vi "Test MQTT-3.3.2-3.vi"(8 "error in (no error)":errorcluster, 11 "Connection Config":refnum<class "Connection.lvclass">) -> (0 "error out":errorcluster, 3 "Connection Config dup":refnum<class "Connection.lvclass">)   [LabVIEW 2013]
uses:
  <vilib>/LabVIEW Open Source Project/MQTT Connection/MQTT_Connection/Connection/Connection.lvclass
  <vilib>/LabVIEW Open Source Project/MQTT Client/Client class/Client.lvclass/Client.ctl
  <vilib>/LabVIEW Open Source Project/MQTT Control Packets/Control Packets/PUBLISH/PUBLISH.lvclass
  <vilib>/addons/_JKI Toolkits/Caraya/classes/Test/Test.lvclass
  <vilib>/LabVIEW Open Source Project/MQTT Client/Client class/Client.lvclass
  <vilib>/addons/_JKI Toolkits/Caraya/classes/Assert/Assert.lvclass
  <vilib>/LabVIEW Open Source Project/MQTT Connection/MQTT_Base/Base Class/MQTT_Base.lvclass
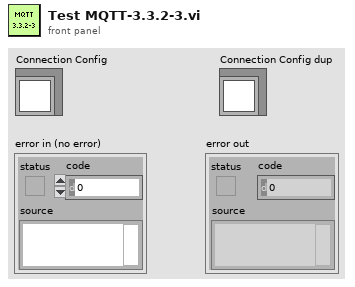
[diagram p1: front panel]
types:
  T1 = typedef "MQTT Client.lvlib/Client.lvclass/Public Events -- cluster.ctl" = cluster{"Connection Status":refnum<user-event>, "Connected":refnum<user-event>, "Application Message":refnum<user-event>}
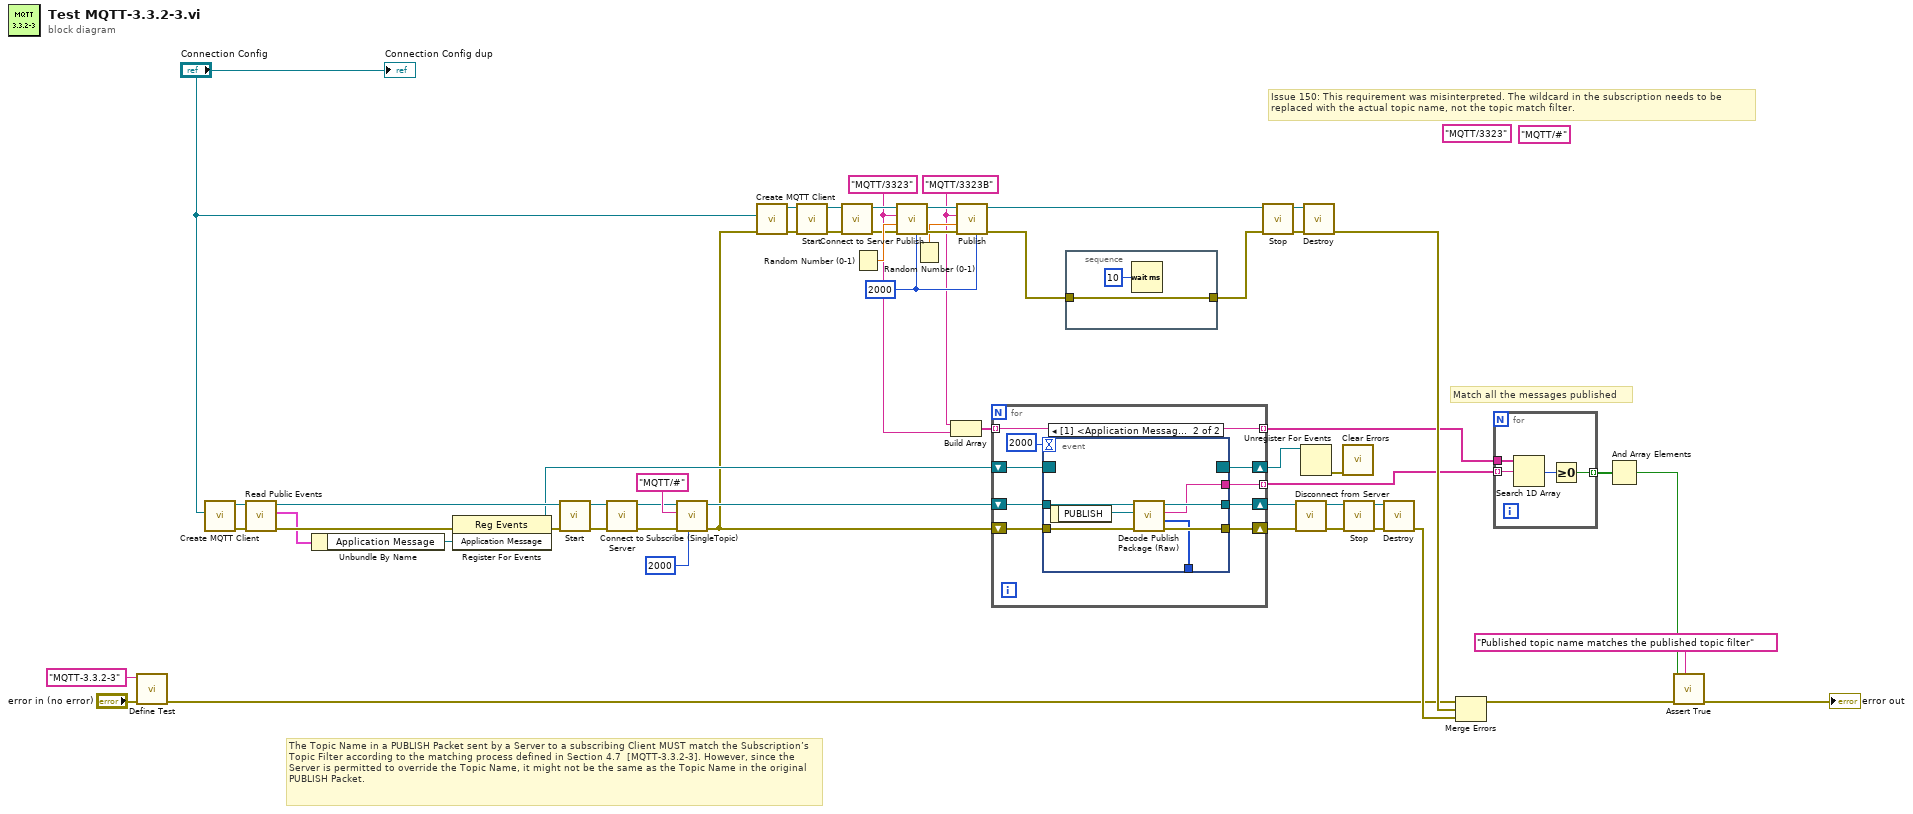
[diagram p0: block diagram]
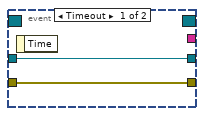
[diagram p2: hidden frame]
diagram:
  w36 = 2000 ("timeout (100ms)")
  w11 = "MQTT/3323B" ("Topic Filter")
  (unwired) "MQTT/3323" ("Topic Filter")
  (unwired) "MQTT/#" ("Topic Filter")
  w10 = "MQTT/3323" ("Topic Filter")
  # "Match all the messages published"
  # "Issue 150: This requirement was misinterpreted. The wildcard in the subscription needs to be\nreplaced with the actual topic name, not the topic match filter."
  # "The Topic Name in a PUBLISH Packet sent by a Server to a subscribing Client MUST match the Subscription’s Topic Filter according to the matching process defined in Section 4.7  [MQTT-3.3.2-3]. However, since the Server is permitted to override the Topic Name, it might not be the same as the Topic Name in the original PUBLISH Packet."
  n1 = call <vilib>:"Define Test.vi"("error in (no error)"="error in (no error)", "Label (VI Title)"="MQTT-3.3.2-3") -> ("error out"=w2:errorcluster)  [unwired: 9 in]
  n2 = call <vilib>:"Create MQTT Client.vi"("Connection Configuration"="Connection Config") -> ("error out"=w30:errorcluster, "Client out"=w29:refnum<class "Client.lvclass">)  [unwired: 9 in]
  n3 = call <vilib>:"Read Public Events.vi"("error in (no error)"=w30, "Client in"=w29) -> ("error out"=w31:errorcluster, "Client Public Events"=w24:T1, "Client out"=w33:refnum<class "Client.lvclass">)  [unwired: 7 in]
  n4 = Unbundle By Name(w24) -> ("Application Message"=w23:refnum<user-event>)
  n5 = register-events(error in=w31, w23) -> (reference out=w8:refnum<event-registration>, error out=w32:errorcluster)  [unwired: 1 in]
  n6 = call <vilib>:"Start.vi"("error in (no error)"=w32, "MQTT_Base in"=w33) -> ("error out"=w26:errorcluster, "MQTT_Base out"=w27:refnum<class "Client.lvclass">)  [unwired: 7 in, 1 out]
  n7 = call <vilib>:"Connect to Server.vi"("error in (no error)"=w26, "Client in"=w27) -> ("error out"=w19:errorcluster, "Client out"=w20:refnum<class "Client.lvclass">)  [unwired: 6 in, 2 out]
  n8 = call <vilib>:"Subscribe (SingleTopic).vi"("timeout (100ms)"=2000, "error in (no error)"=w19, "Topic Filter"="MQTT/#", "MQTT_Base in"=w20) -> ("error out"=w1:errorcluster, "MQTT_Base out"=w9:refnum<class "Client.lvclass">)  [unwired: 5 in, 1 out]
  n9 = call <vilib>:"Create MQTT Client.vi"("error in (no error)"=w1, "Connection Configuration"="Connection Config") -> ("error out"=w44:errorcluster, "Client out"=w45:refnum<class "Client.lvclass">)  [unwired: 8 in]
  n10 = call <vilib>:"Start.vi"("error in (no error)"=w44, "MQTT_Base in"=w45) -> ("error out"=w49:errorcluster, "MQTT_Base out"=w50:refnum<class "Client.lvclass">)  [unwired: 7 in, 1 out]
  n11 = call <vilib>:"Connect to Server.vi"("error in (no error)"=w49, "Client in"=w50) -> ("error out"=w3:errorcluster, "Client out"=w18:refnum<class "Client.lvclass">)  [unwired: 6 in, 2 out]
  n12 = Random Number (0-1)() -> (number: 0 to 1=w48:dbl)
  n13 = call <vilib>:"Publish.vi"("timeout (1000ms)"=w36, "error in (no error)"=w3, "Payload"=w48, "Topic Name (empty: Payload name)"=w10, "Client in"=w18) -> ("error out"=w41:errorcluster, "Client out"=w42:refnum<class "Client.lvclass">)  [unwired: 4 in, 1 out]
  n14 = Random Number (0-1)() -> (number: 0 to 1=w40:dbl)
  n15 = Build Array(w11, w10) -> (w37:string[])
  n16 = call <vilib>:"Publish.vi"("timeout (1000ms)"=w36, "error in (no error)"=w41, "Payload"=w40, "Topic Name (empty: Payload name)"=w11, "Client in"=w42) -> ("error out"=w5:errorcluster, "Client out"=w12:refnum<class "Client.lvclass">)  [unwired: 4 in, 1 out]
  n17 = for {
    shift-right: [w61] -> w17
    shift-left: w8 -> [w62]
    tunnel: [w58] -> w6 mode=indexing
    shift-right: [w63] -> w16
    shift-left: w9 -> [w60]
    shift-right: [w64] -> w13
    shift-left: w1 -> [w59]
    tunnel: w37 -> [w57] mode=indexing
    tunnel: [w57] -> w7 mode=indexing
    n18 = event shown="[1] <Application Message>: User Event" {
      selector: w62 -> [_ _]
      dyn-events: [_ _] -> w61
      timeout: 2000 -> [_ _]
      tunnel: w60 -> [w67 w74]
      tunnel: [w67 w72] -> w63
      tunnel: [w66 w71] -> w64
      tunnel: w59 -> [w66 w70]
      tunnel: [_ w69] -> _
      tunnel: [_ w68] -> w58
      event Timeout {
        n19 = event-data() -> ()  [unwired: 1 in, 1 out]
      }
      event User Event {
        n20 = event-data() -> ("PUBLISH"=w73:refnum<class "PUBLISH.lvclass">)  [unwired: 1 in]
        n21 = call <vilib>:"Decode Publish Package (Raw).vi"("error in (no error)"=w70, "PUBLISH"=w73, "MQTT_Base in"=w74) -> ("error out"=w71:errorcluster, "Payload"=w69:u8[], "Topic"=w68:string, "MQTT_Base out"=w72:refnum<class "Client.lvclass">)  [unwired: 5 in]
      }
    }
  }
  n22 = stacked-sequence {
    tunnel: w5 -> [w76]
    tunnel: [w76] -> w4
    frame #0 {
      n23 = Wait (ms)(milliseconds to wait=u32 10) -> ()  [unwired: 1 out]
    }
  }
  n24 = call <vilib>:"Stop.vi"("error in (no error)"=w4, "MQTT_Base in"=w12) -> ("error out"=w46:errorcluster, "MQTT_Base out"=w47:refnum<class "Client.lvclass">)  [unwired: 7 in, 1 out]
  n25 = call <vilib>:"Disconnect from Server.vi"("error in (no error)"=w13, "Client in"=w16) -> ("error out"=w14:errorcluster, "Client out"=w15:refnum<class "Client.lvclass">)  [unwired: 7 in, 1 out]
  n26 = Unregister For Events(event registration refnum=w17) -> (error out=w43:errorcluster)  [unwired: 1 in]
  n27 = call <vilib>:"Destroy.vi"("error in (no error)"=w46, "MQTT_Base in"=w47) -> ("error out"=w51:errorcluster)  [unwired: 8 in, 1 out]
  n28 = call <vilib>:"Clear Errors.vi"("error in (no error)"=w43) -> ()  [unwired: 6 in, 1 out]
  n29 = call <vilib>:"Stop.vi"("error in (no error)"=w14, "MQTT_Base in"=w15) -> ("error out"=w35:errorcluster, "MQTT_Base out"=w34:refnum<class "Client.lvclass">)  [unwired: 7 in, 1 out]
  n30 = call <vilib>:"Destroy.vi"("error in (no error)"=w35, "MQTT_Base in"=w34) -> ("error out"=w28:errorcluster)  [unwired: 8 in, 1 out]
  n31 = Merge Errors(w2, w51, w28) -> (w52:errorcluster)
  n32 = for {
    tunnel: w6 -> [w79] mode=indexing
    tunnel: w7 -> [w80]
    tunnel: [w77] -> w39 mode=indexing
    n33 = Search 1D Array(1D array=w80, element=w79) -> (index of element=w78:i32)  [unwired: 1 in]
    n34 = Greater Or Equal To 0?(x=w78) -> (x >= 0?=w77:bool)
  }
  n35 = And Array Elements(Boolean array=w39) -> (logical AND=w38:bool)
  n36 = call <vilib>:"Assert True.vi"("Label"="Published topic name matches the published topic filter", "error in (no error)"=w52, "True?"=w38) -> ("error out"=→"error out":errorcluster)  [unwired: 8 in]
  "Connection Config dup" <- "Connection Config"
